vi "CPU_Load.vi"() -> (3 "CPU [%]":dbl)   [LabVIEW 2025]
uses:
  <vilib>/NI_Real-Time Target Support.lvlib
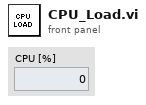
[diagram p1: front panel]
types:
  T1 = typedef "NI_Real-Time Target Support.lvlib/RT CPU Load.ctl" = cluster{"Total (%)":dbl, "Time Critical (%)":dbl, "Timed Structures (%)":dbl, "High (%)":dbl, "Above Normal (%)":dbl, "Normal (%)":dbl, "Background (%)":dbl, "Idle (%)":dbl, "ISR (%)":dbl}
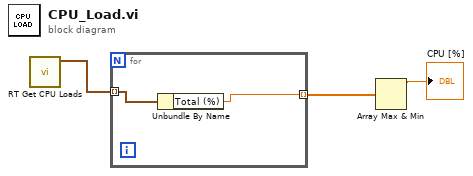
[diagram p0: block diagram]
diagram:
  n1 = call <vilib>:"RT Get CPU Loads.vi"() -> ("CPU loads"=w1:T1[])  [unwired: 10 in, 1 out]
  n2 = for {
    tunnel: w1 -> [w5] mode=indexing
    tunnel: [w4] -> w2 mode=indexing
    n3 = Unbundle By Name(w5) -> ("Total (%)"=w4:dbl)
  }
  n4 = Array Max & Min(array=w2) -> (max value=→"CPU [%]":dbl)  [unwired: 3 out]
